vi "Generate Log Entry.vi"(8 "error in":errorcluster, 11 "Message":string) -> (0 "error out":errorcluster, 3 "Log Entry":T1 {"Time" format="%<%x %.3X>T"})   [LabVIEW 2026]
doc: "Generate log entry using provided message and current time. If the provided error contains an error the error code will be prepended to the message."
uses:
  Type Definitions/Log Entry--cluster.ctl
  <vilib>/Utility/error.llb/DialogType.ctl
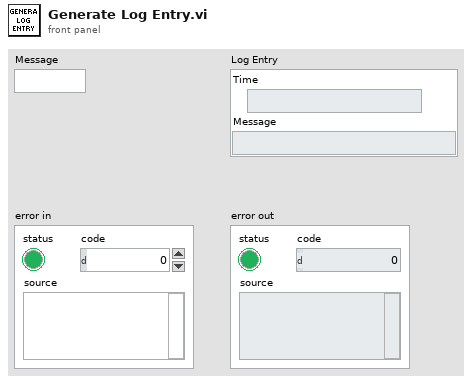
[diagram p1: front panel]
types:
  T1 = typedef "Log Entry--cluster.ctl" = cluster{"Time":timestamp, "Message":string}
  T2 = typedef "DialogType.ctl" = u16
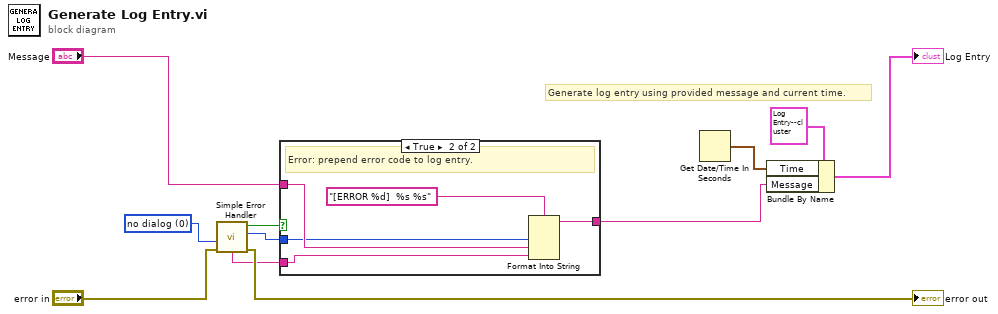
[diagram p0: block diagram]
diagram:
  w7 = T2 0 items=["no dialog", "OK message", "continue or stop message", "OK message + warnings", "continue/stop + warnings"] ("type of dialog (OK msg:1)")
  # "Generate log entry using provided message and current time."
  n1 = call <vilib>:"Simple Error Handler.vi"("type of dialog (OK msg:1)"=w7, "error in (no error)"="error in") -> ("error?"=w6:bool, "code out"=w5:i32, "error out"=→"error out":errorcluster, "message"=w1:string)  [unwired: 3 in, 1 out]
  n2 = case shown="True" w6 {
    tunnel: w5 -> [_ w15]
    tunnel: "Message" -> [w12 w16]
    tunnel: [w12 w14] -> w3
    tunnel: w1 -> [_ w13]
    frame False {
      # "No error"
    }
    frame True {
      # "Error: prepend error code to log entry."
      n3 = Format Into String(format string="[ERROR %d]  %s %s", w15, w16, w13) -> (resulting string=w14:string)  [unwired: 2 in, 1 out]
    }
  }
  n4 = Get Date/Time In Seconds() -> (seconds since 1Jan1904=w10:timestamp)
  n5 = Bundle By Name(cluster=T1 {"Time"=timestamp(0 s since 1904-01-01), "Message"=""} ("Log Entry"), "Time"=w10, "Message"=w3) -> (→"Log Entry":T1)
